vi "_RotatePoints.vi"(9 "Origin":T1, 10 "Angle":dbl, 11 "Points in":T1[](array[typedef])) -> (3 "Points out":T1[](array[typedef]))   [LabVIEW 2020, in "OpenLvVision_Overlays.lvlib"]
uses:
  OpenLvVision_Overlays.lvlib
  TypeDefs/PointI32.ctl
  <vilib>/Analysis/coordinate.llb/2D Cartesian Coordinate Shift (Array).vi
  <vilib>/Analysis/coordinate.llb/2D Cartesian Coordinate Rotation (Array).vi
  <vilib>/Analysis/NI_AALPro.lvlib
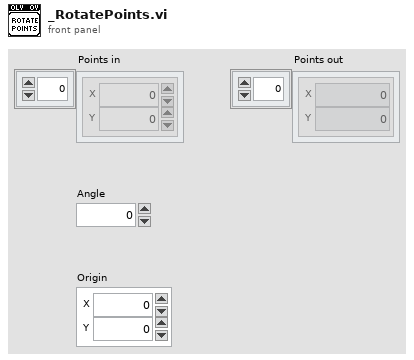
[diagram p1: front panel]
types:
  T1 = typedef "OpenLvVision_Overlays.lvlib/PointI32.ctl" = cluster{"X":i32, "Y":i32}
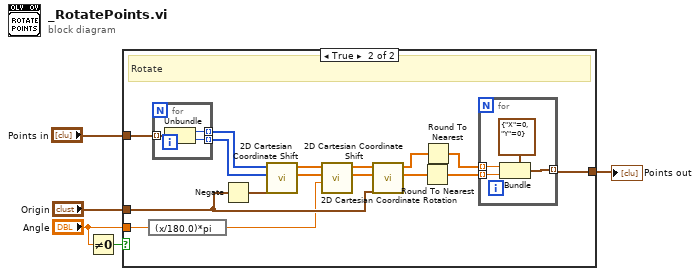
[diagram p0: block diagram]
diagram:
  n1 = Not Equal To 0?(x="Angle") -> (x != 0?=w2:bool)
  n2 = case shown="True" w2 {
    tunnel: "Points in" -> [w6 w18]
    tunnel: "Origin" -> [_ w14]
    tunnel: [w6 w12] -> w3
    tunnel: "Angle" -> [_ w11]
    frame False {
      # "Angle 0"
    }
    frame True {
      # "Rotate"
      n3 = expression code="(x/180.0)*pi" ("degrees to radians")(w11) -> (w13:dbl)
      n4 = for {
        tunnel: w18 -> [w29] mode=indexing
        tunnel: [w28] -> w17 mode=indexing
        tunnel: [w27] -> w16 mode=indexing
        n5 = Unbundle(w29) -> ("X"=w27:i32, "Y"=w28:i32)
      }
      n6 = Negate(x=w14) -> (-x=w15:T1)
      n7 = call-poly <vilib>:"2D Cartesian Coordinate Shift.vi"("shift"=w15, "Y"=w17, "X"=w16) -> ("Y Out"=w21:dbl[], "X Out"=w22:dbl[])  [unwired: 6 in, 1 out]
      n8 = call-poly <vilib>:"2D Cartesian Coordinate Rotation.vi"("theta"=w13, "Y"=w21, "X"=w22) -> ("Y Out"=w19:dbl[], "X Out"=w20:dbl[])  [unwired: 6 in, 1 out]
      n9 = call-poly <vilib>:"2D Cartesian Coordinate Shift.vi"("shift"=w14, "Y"=w19, "X"=w20) -> ("Y Out"=w9:dbl[], "X Out"=w10:dbl[])  [unwired: 6 in, 1 out]
      n10 = Round To Nearest(number=w9) -> (nearest integer value=w7:dbl[])
      n11 = Round To Nearest(number=w10) -> (nearest integer value=w8:dbl[])
      n12 = for {
        tunnel: w8 -> [w26] mode=indexing
        tunnel: w7 -> [w25] mode=indexing
        tunnel: [w24] -> w12 mode=indexing
        n13 = Bundle(cluster=T1 {"X"=0, "Y"=0} ("Origin"), "X"=w26, "Y"=w25) -> (w24:T1)
      }
    }
  }
  "Points out" <- w3
